vi "Caller2.vi"(11 "error in":errorcluster) -> (15 "error out":errorcluster)   [LabVIEW 2026]
doc: "Issue 136 enum example: a Level typedef constant at High, the last item."
uses:
  Level.ctl
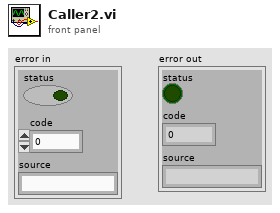
[diagram p1: front panel]
types:
  T1 = typedef "Level.ctl" = enum16{"Low", "Mid", "High"}
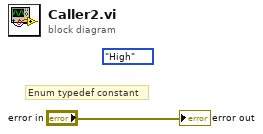
[diagram p0: block diagram]
diagram:
  (unwired) Level."High" ("Level")
  # "Enum typedef constant"
  "error out" <- "error in"
